vi "Synchronize Palette with Directory.vi"() -> ()   [LabVIEW 2020]
uses:
  source/Package/PackageFile.lvclass
panel:
  out "error out":errorcluster
  in  "error in (no error)":errorcluster
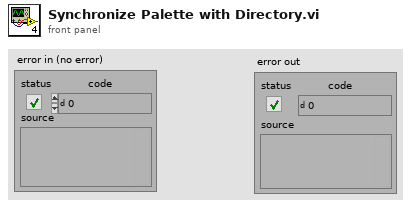
[diagram p1: front panel]
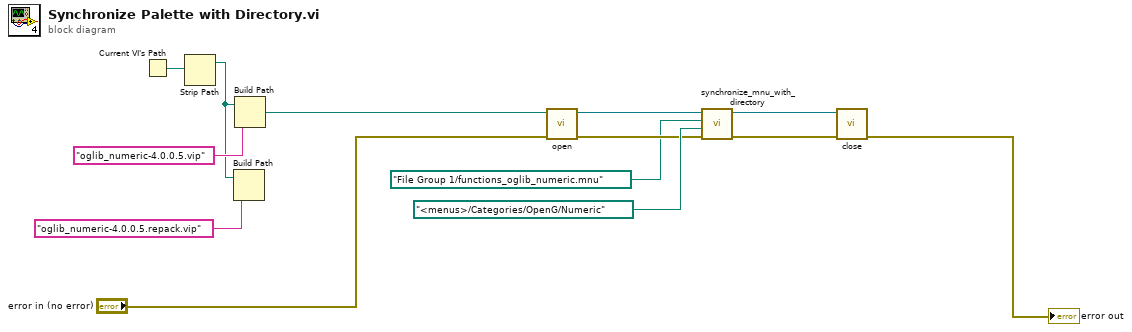
[diagram p0: block diagram]
diagram:
  n1 = Current VI's Path() -> (path=w13:path)
  n2 = Strip Path(path=w13) -> (stripped path=w9:path)  [unwired: 1 out]
  n3 = Build Path(base path=w9, name or relative path="oglib_numeric-4.0.0.5.repack.vip") -> ()  [unwired: 1 out]
  n4 = Build Path(base path=w9, name or relative path="oglib_numeric-4.0.0.5.vip") -> (appended path=w11:path)
  n5 = call "open.vi"("error in"="error in (no error)", "Package File Path"=w11) -> ("error out"=w5:errorcluster, "PackageFile out"=w2:refnum<class "PackageFile.lvclass">)  [unwired: 8 in]
  n6 = call "synchronize_mnu_with_directory.vi"("error in (no error)"=w5, "Synchronized Directory"=path "<menus>/Categories/OpenG/Numeric" ("Unpacked File"), "MNU File"=path "File Group 1/functions_oglib_numeric.mnu" ("Unpacked File"), "PackageFile in"=w2) -> ("error out"=w4:errorcluster, "PackageFile out"=w1:refnum<class "PackageFile.lvclass">)  [unwired: 6 in]
  n7 = call "close.vi"("error in (no error)"=w4, "PackageFile in"=w1) -> ("error out"=→"error out":errorcluster)  [unwired: 8 in, 1 out]
